vi "to_item.vi"(8 "error in (no error)":errorcluster, 11 "Table in":refnum<class "InlineTable.lvclass">) -> (0 "error out":errorcluster, 3 "Item out":refnum<class "Item.lvclass">)   [LabVIEW 2020, in "toml_edit.lvlib" / "InlineTable.lvclass"]
uses:
  InlineTable.lvclass
  Item/Item.lvclass
  InlineTable.lvclass/InlineTable.ctl
  dragon_toml_64.dll
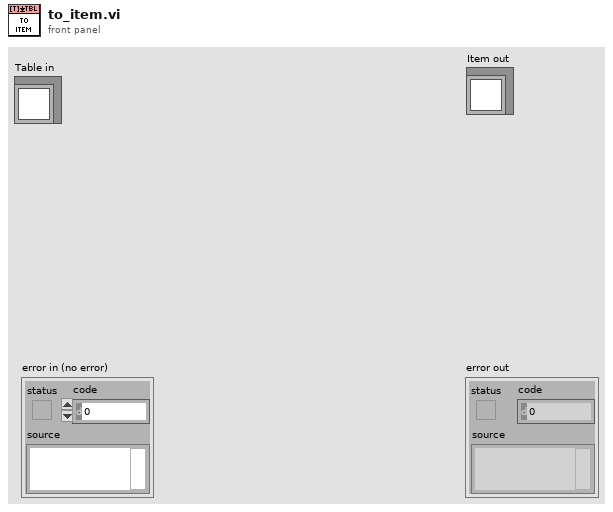
[diagram p1: front panel]
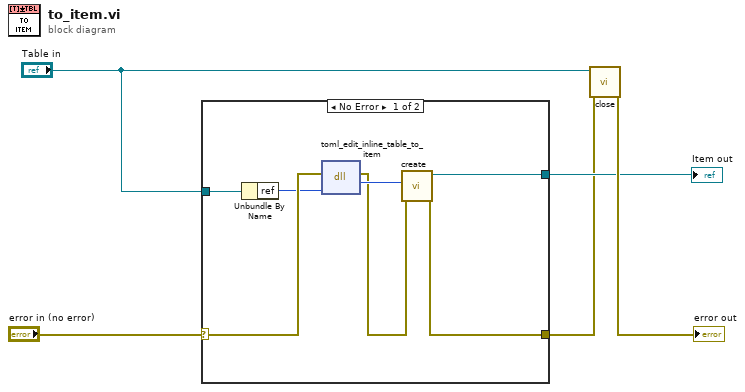
[diagram p0: block diagram]
diagram:
  n1 = case shown="No Error" "error in (no error)" {
    selector: "error in (no error)" -> [w12 w13]
    tunnel: "Table in" -> [w11 _]
    tunnel: [w10 _] -> w2
    tunnel: [w6 w13] -> w1
    frame No Error {
      n2 = Unbundle By Name(w11) -> ("ref"=w8:u64)
      n3 = dll-call lib="C:/projects/dragon-desktop/source/submodules/toml-edit-labview/lv_src/dragon_toml_*.dll" fn="toml_edit_inline_table_to_item"(error in=w12, "table_ref"=w8) -> (error out=w7:errorcluster, "item_ref"=w9:u64)  [unwired: 3 in, 1 out]
      n4 = call "create.vi"("error in (no error)"=w7, "ref"=w9) -> ("error out"=w6:errorcluster, "Item out"=w10:refnum<class "Item.lvclass">)  [unwired: 7 in, 1 out]
    }
    frame Error {
    }
  }
  "Item out" <- w2
  n5 = call "close.vi"("error in (no error)"=w1, "Table in"="Table in") -> ("error out"=→"error out":errorcluster)  [unwired: 9 in]
